vi "CIF Receive.vi"(8 "error in (no error)":errorcluster, 9 "Timoeut ms":u32, 10 "Data In":u8[](array[numeric]), 11 "Subscriber Reference":T3 {"refnum" format="%.0x"}) -> (0 "error out":errorcluster, 1 "Array Length":u32, 2 "Data Out":u8[](array[numeric]), 3 "CIF Channel Header":T2, 4 "Timeout":bool, 5 "CIF Subscriber Stats":T1)   [LabVIEW 2021, in "Iceoryx.lvlib"]
doc: "Read from an iceoryx CIF pcap queue. \n\n<B>Data In:</B> Memory location to accept the flattened PCAP formatted data of the correct Link Type. \n<B>Data Out:</B> The flattened PCAP formatted data from the queue.\n<B>Array Length:</B> The length of valid bytes that were copied into the Data Out buffer. Note, this will be 48 smaller than the Length of the CIF Channel Header as it also includes the header data."
uses:
  Iceoryx.lvlib
  Refnum/Typedef/CIF Subscriber Refnum.ctl
  typedef/CIF Channel Header.ctl
  typedef/CIF Pcap Subscriber Stats.ctl
  SubVIs/Convert Error Core.vi
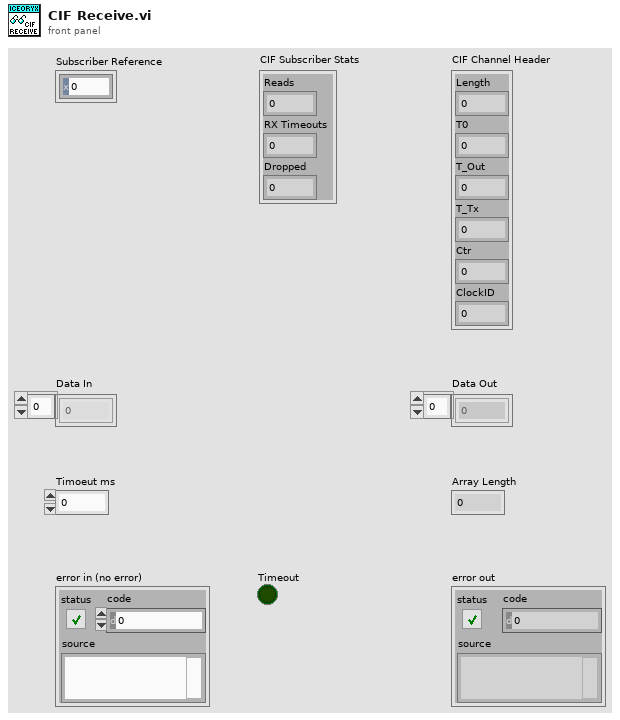
[diagram p1: front panel]
types:
  T1 = typedef "Iceoryx.lvlib/CIF Pcap Subscriber Stats.ctl" = cluster{"Reads":u64, "RX Timeouts":u64, "Dropped":u64}
  T2 = typedef "Iceoryx.lvlib/CIF Channel Header.ctl" = cluster{"Length":u64, "T0":i64, "T_Out":i64, "T_Tx":i64, "Ctr":u64, "ClockID":u8}
  T3 = typedef "Iceoryx.lvlib/CIF Subscriber Refnum.ctl" = cluster{"refnum":u64, "CIF Sub":enum8{"cifsub"}}
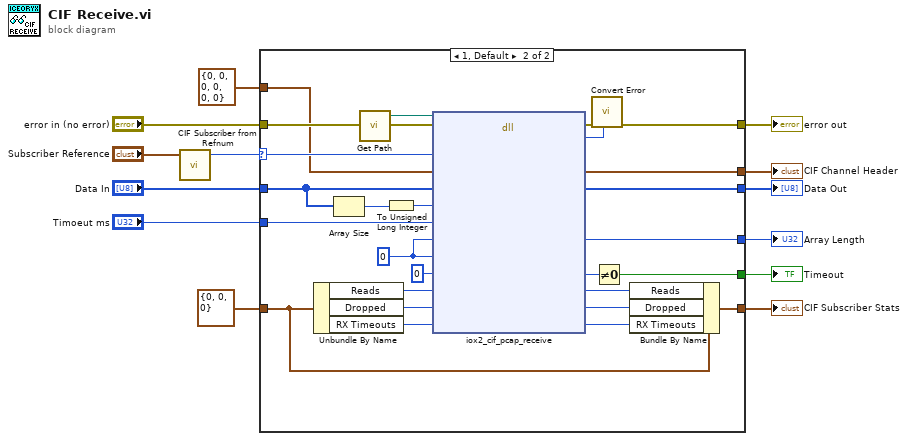
[diagram p0: block diagram]
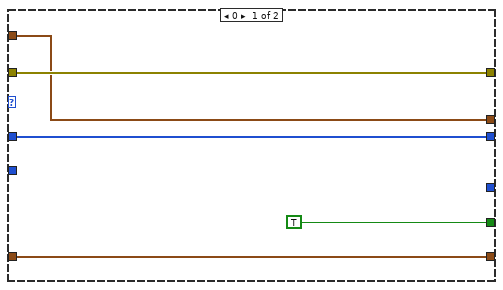
[diagram p2: hidden frame]
diagram:
  n1 = call "CIF Subscriber from Refnum.vi"("CIF Subscriber Refnum"="Subscriber Reference") -> ("CIF Subscriber U64"=w1:u64)  [unwired: 4 in]
  n2 = case shown="1, Default" w1 {
    selector: w1 -> [_ w38]
    tunnel: "error in (no error)" -> [w18 w44]
    tunnel: "Data In" -> [w17 w34]
    tunnel: [w17 w43] -> w6
    tunnel: [w18 w39] -> w12
    tunnel: [_ w20] -> w10
    tunnel: "Timoeut ms" -> [_ w37]
    tunnel: [TRUE w35] -> w8
    tunnel: T2 {"Length"=0, "T0"=0, "T_Out"=0, "T_Tx"=0, "Ctr"=0, "ClockID"=0} ("CIF Channel Header") -> [w14 w32]
    tunnel: [w14 w31] -> w4
    tunnel: T1 {"Reads"=0, "RX Timeouts"=0, "Dropped"=0} ("CIF Subscriber Stats") -> [w15 w27]
    tunnel: [w15 w23] -> w2
    frame 0 {
    }
    frame 1, Default {
      w21 = u32 0 ("actual")
      n3 = Unbundle By Name(w27) -> ("Reads"=w30:u64, "Dropped"=w28:u64, "RX Timeouts"=w29:u64)
      n4 = Array Size(array=w34) -> (size(s)=w33:i32)
      n5 = call "Get Path.vi"() -> ("libiox2_cif path"=w42:path)  [unwired: 4 in]
      n6 = To Unsigned Long Integer(number=w33) -> (unsigned 32bit integer=w22:u32)
      n7 = dll-call lib="D:/dev/iceoryx2_lvwrapper/dist/iox2_cif.dll" fn="iox2_cif_pcap_receive"(path in=w42, error in=w44, "subscriber"=w38, "header"=w32, "pcap"=w34, "cap"=w22, "timeout"=w37, "actual"=w21, "max"=w21, "timed_out"=0, "samples"=w30, "dropped"=w28, "timeouts"=w29) -> (error out=w41:errorcluster, "return type"=w40:i32, "header"=w31:T2, "pcap"=w43:u8[], "actual"=w20:u32, "timed_out"=w36:i32, "samples"=w26:u64, "dropped"=w24:u64, "timeouts"=w25:u64)  [unwired: 5 in, 1 out]
      n8 = call "Convert Error.vi"("return type"=w40, "error in (no error)"=w41) -> ("error out"=w39:errorcluster)  [unwired: 9 in]
      n9 = Not Equal To 0?(x=w36) -> (x != 0?=w35:bool)
      n10 = Bundle By Name(cluster=w27, "Reads"=w26, "Dropped"=w24, "RX Timeouts"=w25) -> (w23:T1)
    }
  }
  "error out" <- w12
  "Array Length" <- w10
  "Timeout" <- w8
  "Data Out" <- w6
  "CIF Channel Header" <- w4
  "CIF Subscriber Stats" <- w2
